vi "Table Buffer - Flush.vi"(8 "error in (no error)":errorcluster) -> (0 "error out":errorcluster)   [LabVIEW 2025, in "I2C Bus Monitor UI.lvlib"]
uses:
  I2C Bus Monitor UI.lvlib
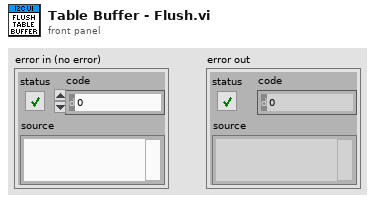
[diagram p1: front panel]
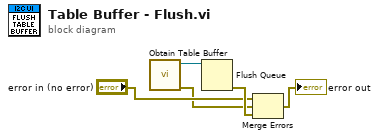
[diagram p0: block diagram]
diagram:
  n1 = call "Obtain Table Buffer.vi"() -> ("error out"=w1:errorcluster, "Table Queue"=w3:refnum<queue>)  [unwired: 10 in]
  n2 = Flush Queue(queue=w3) -> (error out=w4:errorcluster)  [unwired: 1 in, 2 out]
  n3 = Merge Errors("error in (no error)", w1, w4) -> (→"error out":errorcluster)
